vi "Discretization_DiscretizeAQTaylor.vi"(6 "dT_Seconds":dbl, 9 "ContQ":T1, 10 "ContA":T1, 11 "States":i32) -> (0 "Error":bool, 1 "DiscQ":T1, 3 "DiscA":T1)   [LabVIEW 2019, in "Trajectory_Library.lvlib"]
doc: "Discretizes the given continuous A and Q matrices.\n \nRather than solving a 2N x 2N matrix exponential like in DiscretizeQ() (which is expensive), we take advantage of the structure of the block matrix of A and Q.\n \nThe exponential of A*t, which is only N x N, is relatively cheap. 2) The upper-right quarter of the 2N x 2N matrix, which we can approximate using a taylor series to several terms and still be substantially cheaper than taking the big exponential.\n \nInputs:\n - States -- the number of states.\n - contA -- Continuous system matrix.\n - contQ -- Continuous process noise covariance matrix.\n - dtSeconds -- Discretization timestep.\n\nOutputs:\n - DiscA -- the discrete system matrix\n - DiscQ -- process noise covariance matrix.\n - error -- If TRUE, an error occured."
uses:
  Trajectory_Library.lvlib
  <vilib>/Analysis/NI_AALPro.lvlib
  <vilib>/Analysis/7linalg.llb/Real Transpose Matrix.vi
  <vilib>/Analysis/Matrix/NI_Matrix.lvlib
  <vilib>/Analysis/Matrix/Numeric/Add/Add - RM,RM.vi
  <vilib>/Analysis/Matrix/Numeric/Multiply/Multiply - RM,R.vi
  <vilib>/Analysis/NI_AALBase.lvlib
  <vilib>/Analysis/baseanly.llb/Real A x B.vi
  <vilib>/Analysis/Matrix/Datatypes/RealMatrix.ctl
panel:
  # "<States,States>"
  # "<States,States>"
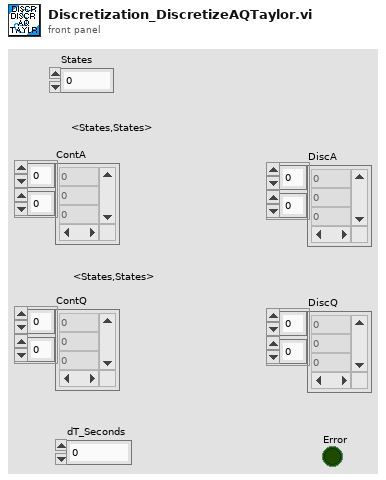
[diagram p1: front panel]
types:
  T1 = typedef "NI_Matrix.lvlib/RealMatrix.ctl" = dbl[][]
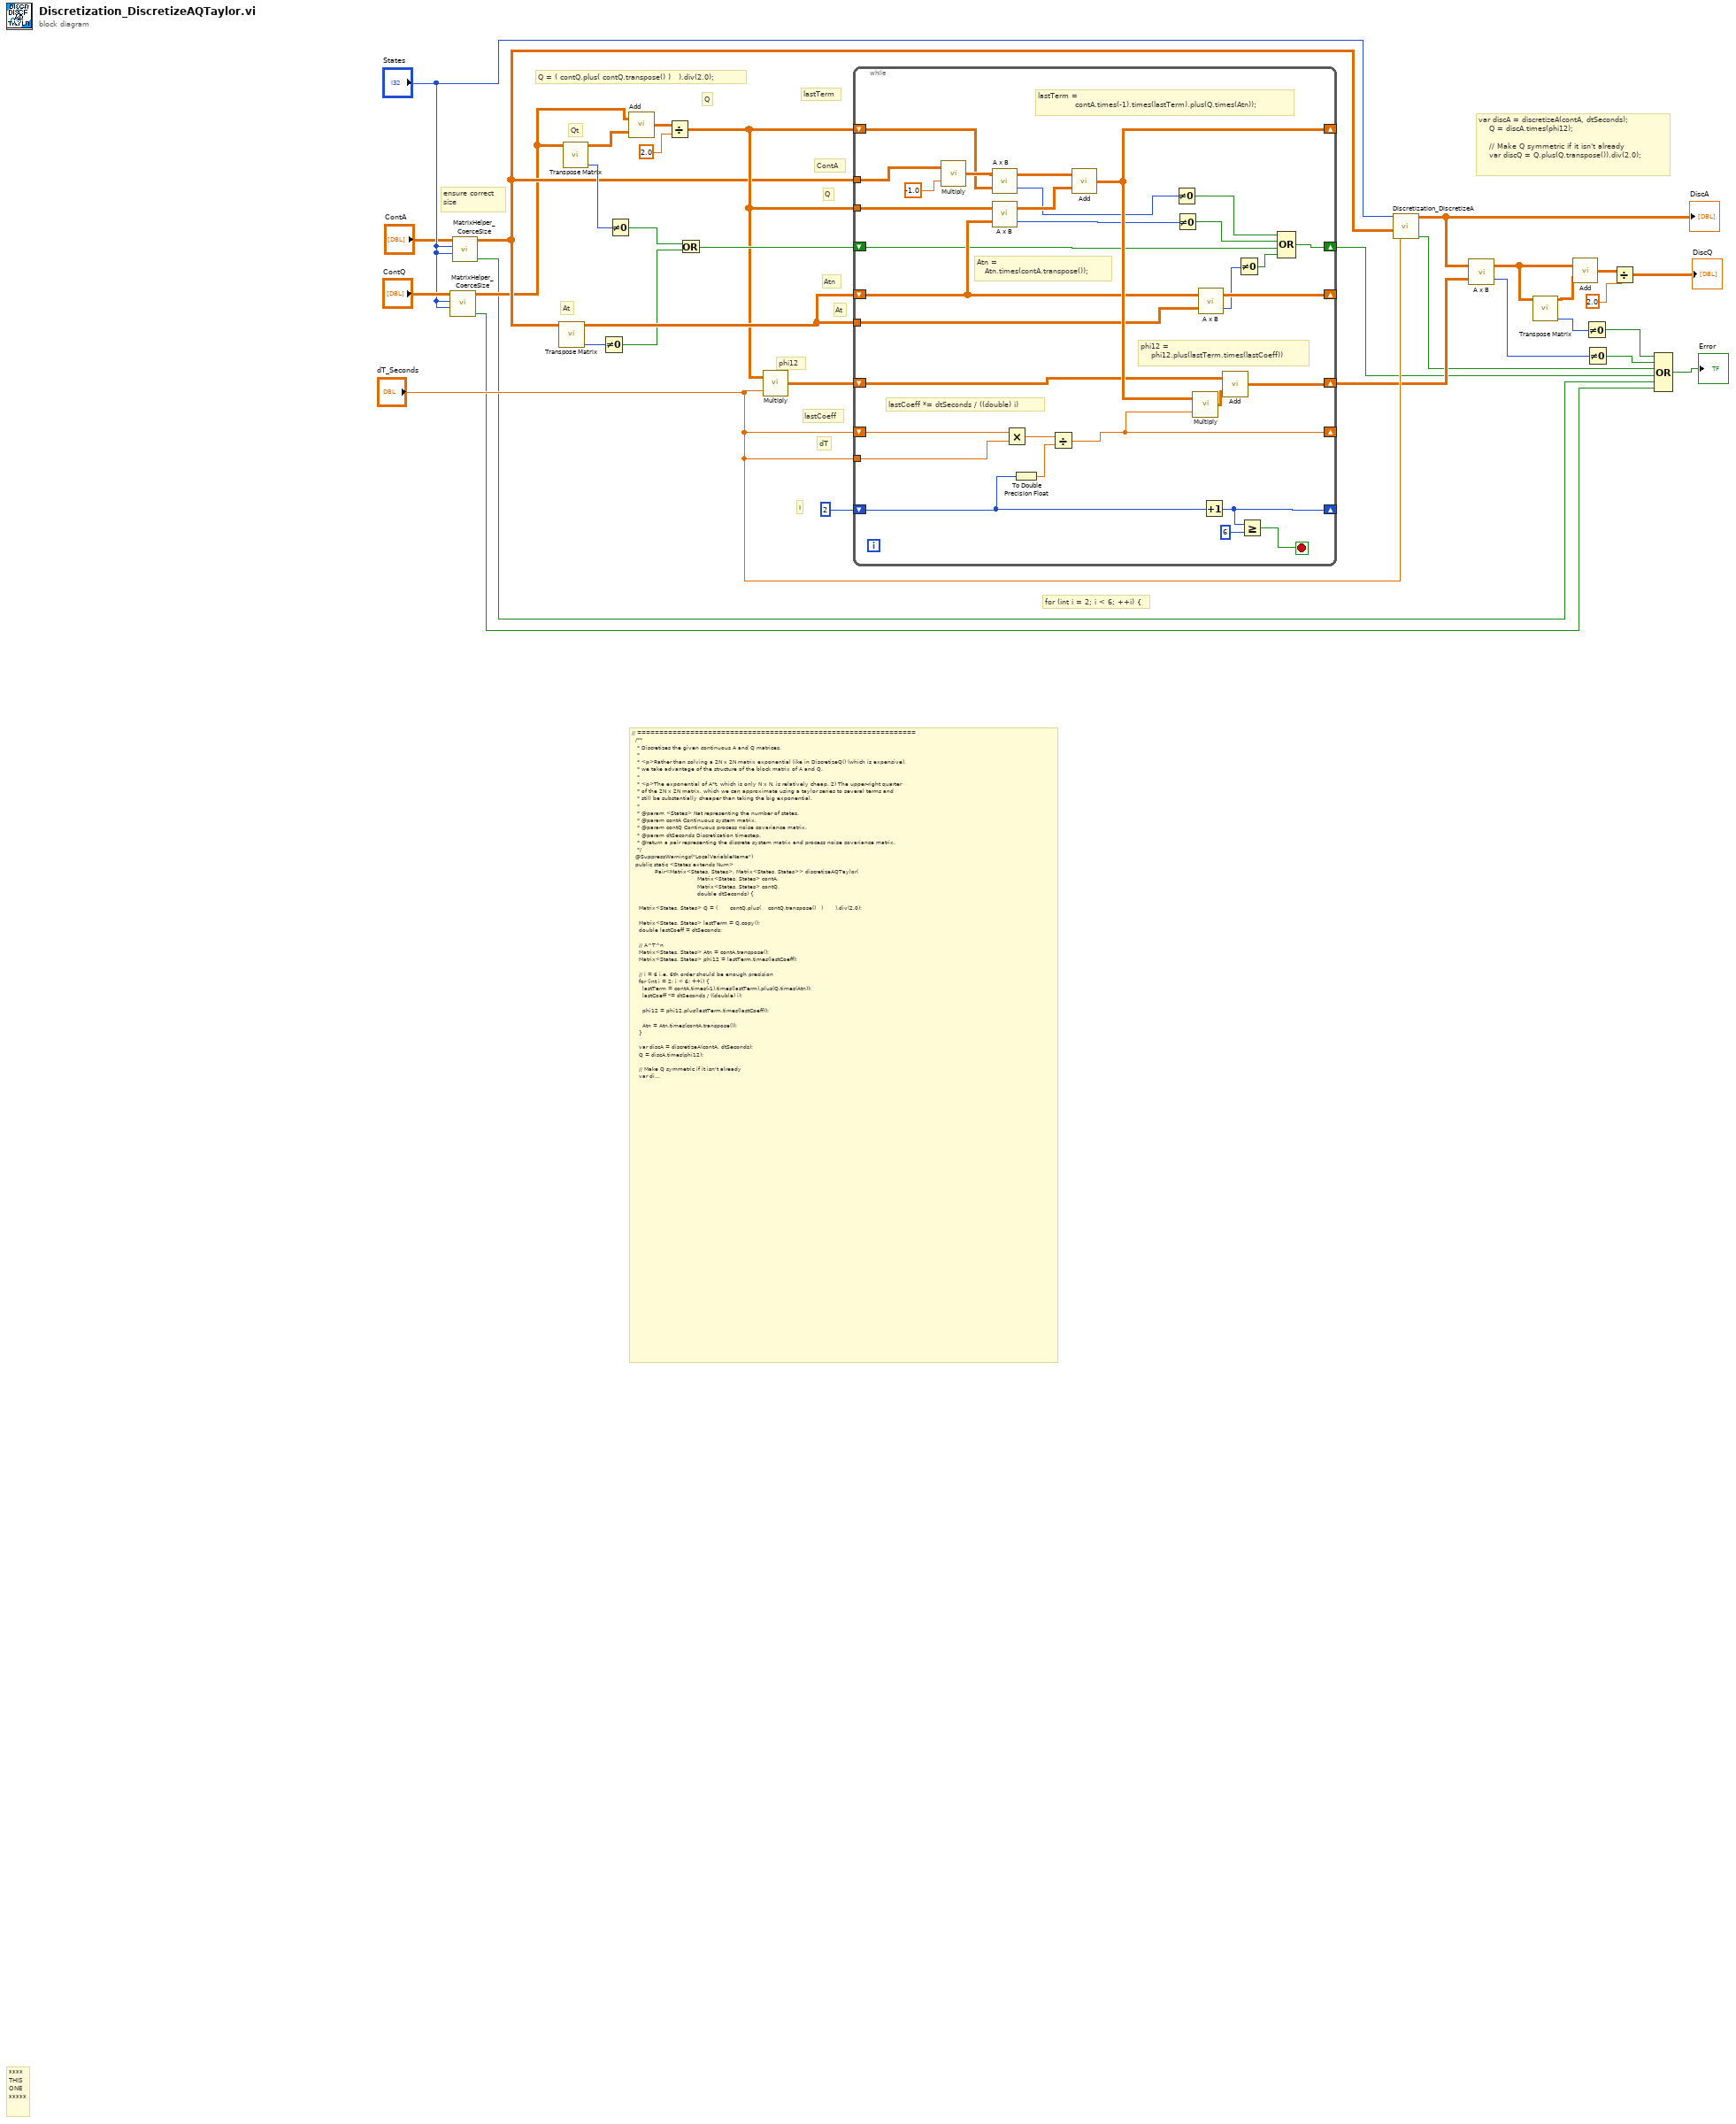
[diagram p0: block diagram]
diagram:
  # "var discA = discretizeA(contA, dtSeconds);\n    Q = discA.times(phi12);\n\n    // Make Q symmetric if it isn't already\n    var discQ = Q.plus(Q.transpose()).div(2.0);"
  # "Q"
  # "dT"
  # "At"
  # "ContA"
  # "for (int i = 2; i < 6; ++i) {"
  # "Atn"
  # "I"
  # "phi12"
  # "Qt"
  # "At"
  # "lastCoeff"
  # "lastTerm"
  # "Q"
  # "Q = ( contQ.plus( contQ.transpose() )   ).div(2.0);"
  # "// ===============================================================\n  /**\n   * Discretizes the given continuous A and Q matrices.\n   *\n   * <p>Rather than solving a 2N x 2N matrix exponential like in DiscretizeQ() (which is expensive),\n   * we take advantage of the structure of the block matrix of A and Q.\n   *\n   * <p>The exponential of A*t, which is only N x N, is relatively cheap. 2) The upper-right quarter\n   * of the 2N x 2N matrix, which we can approximate using a taylor series to several terms and\n   * still be substantially cheaper than taking the big exponential.\n   *\n   * @param <States> Nat representing the number of states.\n   * @param contA Continuous system matrix.\n   * @param contQ Continuous process noise covariance matrix.\n   * @param dtSeconds Discretization timestep.\n   * @return a pair representing the discrete system matrix and process noise covariance matrix.\n   */\n  @SuppressWarnings(\"LocalVariableName\")\n  public static <States extends Num>\n             Pair<Matrix<States, States>, Matrix<States, States>> discretizeAQTaylor(\n                                     Matrix<States, States> contA, \n                                     Matrix<States, States> contQ, \n                                     double dtSeconds) {\n\n    Matrix<States, States> Q = (       contQ.plus(    contQ.transpose()   )       ).div(2.0);\n\n    Matrix<States, States> lastTerm = Q.copy();\n    double lastCoeff = dtSeconds;\n\n    // A^T^n\n    Matrix<States, States> Atn = contA.transpose();\n    Matrix<States, States> phi12 = lastTerm.times(lastCoeff);\n\n    // i = 6 i.e. 6th order should be enough precision\n    for (int i = 2; i < 6; ++i) {\n      lastTerm = contA.times(-1).times(lastTerm).plus(Q.times(Atn));\n      lastCoeff *= dtSeconds / ((double) i);\n\n      phi12 = phi12.plus(lastTerm.times(lastCoeff));\n\n      Atn = Atn.times(contA.transpose());\n    }\n\n    var discA = discretizeA(contA, dtSeconds);\n    Q = discA.times(phi12);\n\n    // Make Q symmetric if it isn't already\n    var discQ = Q.plus(Q.transpose()).div(2.0);\n\n    return new Pair<>(discA, discQ);\n  }"
  # "ensure correct\nsize"
  # "****\nTHIS\nONE\n*****"
  n1 = call "MatrixHelper_CoerceSize.vi"("Columns"="States", "Rows"="States", "input matrix"="ContQ") -> ("Coerced"=w4:bool, "output matrix"=w5:T1)  [unwired: 7 in]
  n2 = call "MatrixHelper_CoerceSize.vi"("Columns"="States", "Rows"="States", "input matrix"="ContA") -> ("Coerced"=w3:bool, "output matrix"=w6:T1)  [unwired: 7 in]
  n3 = call-poly <vilib>:"Transpose Matrix.vi"("Input Matrix"=w6) -> ("error"=w21:i32, "Matrix Transpose"=w29:T1)  [unwired: 9 in]
  n4 = call-poly <vilib>:"Transpose Matrix.vi"("Input Matrix"=w5) -> ("error"=w20:i32, "Matrix Transpose"=w34:T1)  [unwired: 9 in]
  n5 = Not Equal To 0?(x=w21) -> (x != 0?=w18:bool)
  n6 = Not Equal To 0?(x=w20) -> (x != 0?=w19:bool)
  n7 = call-poly <vilib>:"Add.vi"("Real Matrix B"=w34, "Real Matrix A"=w5) -> ("A + B"=w33:T1)
  n8 = Divide(x=w33, y=2.0) -> (x/y=w11:T1)
  n9 = Or(x=w19, y=w18) -> (x .or. y?=w17:bool)
  n10 = call-poly <vilib>:"Multiply.vi"("Real Scalar c"="dT_Seconds", "Real Matrix A"=w11) -> ("A * c"=w30:T1)
  n11 = while {
    shift-right: [w54] -> _
    shift-left: w11 -> [w63]
    shift-right: [w55] -> _
    shift-left: "dT_Seconds" -> [w59]
    shift-right: [w45] -> _
    shift-left: 2 -> [w46]
    tunnel: w6 -> [w47]
    tunnel: w11 -> [w62]
    tunnel: "dT_Seconds" -> [w58]
    shift-right: [w51] -> w10
    shift-left: w30 -> [w53]
    shift-right: [w48] -> _
    shift-left: w29 -> [w50]
    tunnel: w29 -> [w49]
    shift-right: [w42] -> w2
    shift-left: w17 -> [w41]
    stop <- w43 stop-if-true
    # "Atn = \n   Atn.times(contA.transpose());"
    # "phi12 = \n    phi12.plus(lastTerm.times(lastCoeff))"
    # "lastCoeff *= dtSeconds / ((double) i)"
    # "lastTerm = \n              contA.times(-1).times(lastTerm).plus(Q.times(Atn));"
    n12 = call-poly <vilib>:"Multiply.vi"("Real Scalar c"=-1.0, "Real Matrix A"=w47) -> ("A * c"=w64:T1)
    n13 = call-poly <vilib>:"A x B.vi"("B"=w63, "A"=w64) -> ("error"=w40:i32, "A x B"=w61:T1)
    n14 = call-poly <vilib>:"A x B.vi"("B"=w50, "A"=w62) -> ("error"=w39:i32, "A x B"=w60:T1)
    n15 = Multiply(x=w59, y=w58) -> (x*y=w57:dbl)
    n16 = To Double Precision Float(number=w46) -> (double precision float=w56:dbl)
    n17 = Divide(x=w57, y=w56) -> (x/y=w55:dbl)
    n18 = call-poly <vilib>:"Add.vi"("Real Matrix B"=w60, "Real Matrix A"=w61) -> ("A + B"=w54:T1)
    n19 = Not Equal To 0?(x=w40) -> (x != 0?=w35:bool)
    n20 = Not Equal To 0?(x=w39) -> (x != 0?=w36:bool)
    n21 = call-poly <vilib>:"Multiply.vi"("Real Scalar c"=w55, "Real Matrix A"=w54) -> ("A * c"=w52:T1)
    n22 = call-poly <vilib>:"A x B.vi"("B"=w49, "A"=w50) -> ("error"=w37:i32, "A x B"=w48:T1)
    n23 = Increment(x=w46) -> (x+1=w45:i32)
    n24 = call-poly <vilib>:"Add.vi"("Real Matrix B"=w52, "Real Matrix A"=w53) -> ("A + B"=w51:T1)
    n25 = Not Equal To 0?(x=w37) -> (x != 0?=w38:bool)
    n26 = Greater Or Equal?(x=w45, y=6) -> (x >= y?=w43:bool)
    n27 = Compound Arithmetic op=OR(w35, w36, w41, w38) -> (w42:bool)
  }
  n28 = call "Discretization_DiscretizeA.vi"("dT_Seconds"="dT_Seconds", "ContA"=w6, "States"="States") -> ("Error"=w1:bool, "DiscA"=w27:T1)  [unwired: 7 in]
  "DiscA" <- w27
  n29 = call-poly <vilib>:"A x B.vi"("B"=w10, "A"=w27) -> ("error"=w15:i32, "A x B"=w26:T1)
  n30 = call-poly <vilib>:"Transpose Matrix.vi"("Input Matrix"=w26) -> ("error"=w16:i32, "Matrix Transpose"=w25:T1)  [unwired: 9 in]
  n31 = call-poly <vilib>:"Add.vi"("Real Matrix B"=w25, "Real Matrix A"=w26) -> ("A + B"=w24:T1)
  n32 = Not Equal To 0?(x=w16) -> (x != 0?=w13:bool)
  n33 = Not Equal To 0?(x=w15) -> (x != 0?=w14:bool)
  n34 = Divide(x=w24, y=2.0) -> (x/y=→"DiscQ":T1)
  n35 = Compound Arithmetic op=OR(w13, w14, w1, w2, w3, w4) -> (→"Error":bool)
